vi "Create Palette File for VI Folder.vi"(5 "Include VIs in LLBs (T)":bool=TRUE, 6 "Filter Options":T1={"Exclude Dir Name pattern(s)"="^_", "Exclude LLB Name pattern(s)"="^_", "Exclude VI Name pattern(s)"="^_"}, 7 "Palette Icon":picture, 8 "error in":errorcluster, 9 "sub-palettes":path[](array[path]), 10 "Directory Path":path, 11 "Palette File in":path) -> (0 "error out":errorcluster, 2 "dup Directory Path":path, 3 "dup Palette File":path)   [LabVIEW 2014, in "VIHelpeksAPI.lvlib"]
doc: "::: VI Helpeks :::\nCopyright (c) 2000-2026 Konstantin Shifershteyn. All rights reserved."
uses:
  VIHelpeksAPI.lvlib
  <vilib>/Palette API/Palette Menu/Public Type Define/Palette Data.ctl
  <vilib>/Palette API/Palette Menu/Public Type Define/View Format.ctl
  <vilib>/Palette API/Palette Menu/Public Type Define/Items.ctl
  <vilib>/Palette API/Palette Menu/Public Type Define/Item.ctl
  <vilib>/Palette API/Palette Menu/Public Type Define/Help Info.ctl
  <vilib>/Palette API/Palette Menu/Public Type Define/Synchronize Info.ctl
  <vilib>/Palette API/Palette Menu/Public Type Define/Palette type.ctl
  <vilib>/Palette API/Palette Menu/Palette Menu.lvlib
panel:
  # "VI Helpeks\nCopyright (c) 2012-2026 Konstantin Shifershteyn"
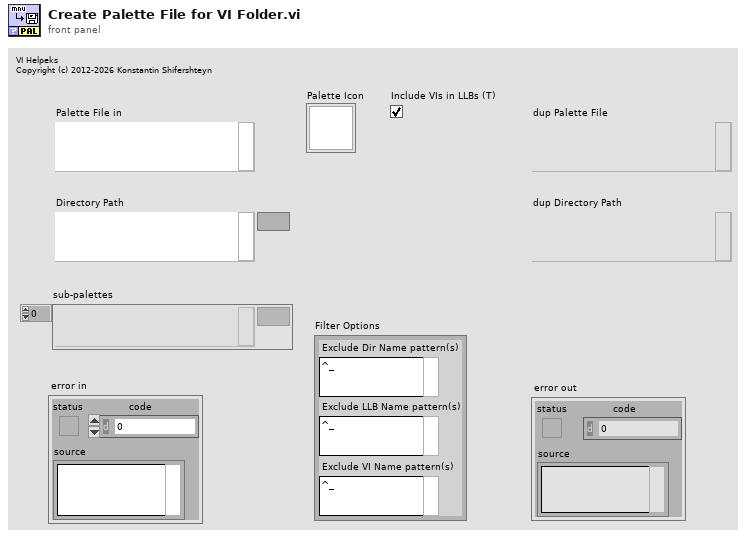
[diagram p1: front panel]
types:
  T1 = cluster{"Exclude Dir Name pattern(s)":string, "Exclude LLB Name pattern(s)":string, "Exclude VI Name pattern(s)":string}
  T2 = typedef "Palette Menu.lvlib/View Format.ctl" = u16
  T3 = typedef "Palette Menu.lvlib/Palette type.ctl" = i32
  T4 = typedef "Palette Menu.lvlib/Palette Data.ctl" = cluster{"display name":string, "view format":T2, "palette width":i16, "items":T5, "256 color icon":picture, "B&W color icon":picture, "help information":T7, "palette description":string, "synchronize information":T8}
  T5 = typedef "Palette Menu.lvlib/Items.ctl" = T6[]
  T6 = typedef "Palette Menu.lvlib/Item.ctl" = cluster{"item path":path, "library path (.lvlib)":path, "use default lvlib palette":bool, "short name":string, "place VI contents":bool, "hide synchronized item":bool, "reserve spot for synch item":bool, "configure when placing VI contents":bool}
  T7 = typedef "Palette Menu.lvlib/Help Info.ctl" = cluster{"help tag":string, "help file path ":path}
  T8 = typedef "Palette Menu.lvlib/Synchronize Info.ctl" = cluster{"synchronize with directory":bool, "synchronize directory path":path}
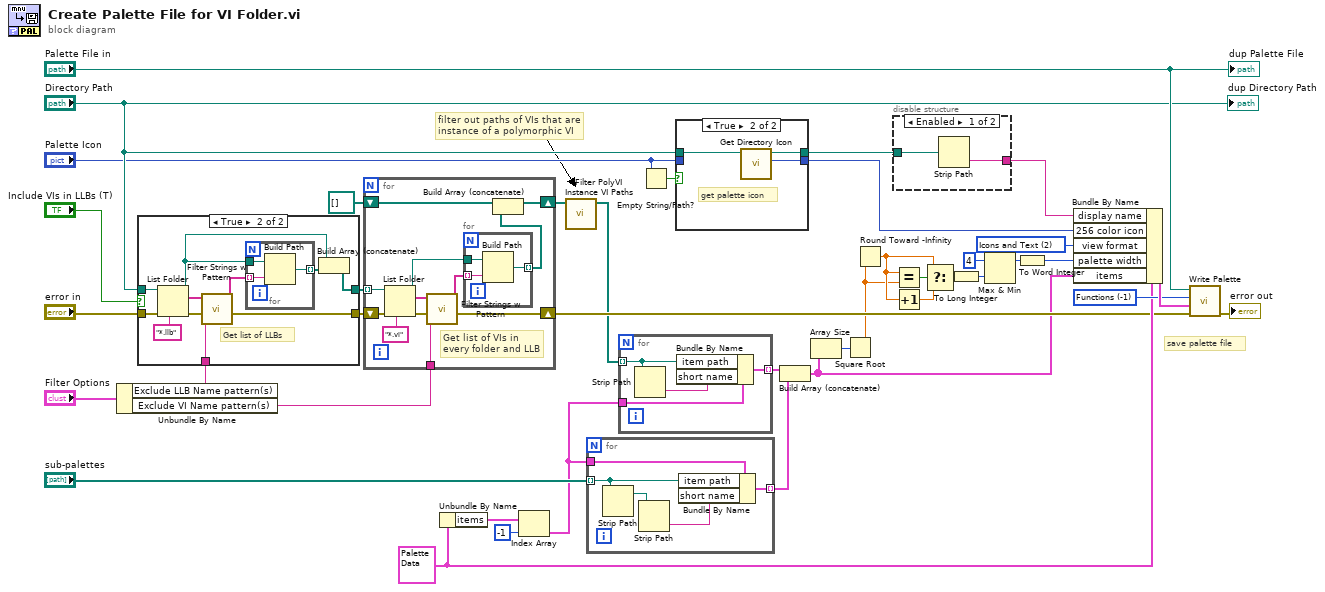
[diagram p0: block diagram]
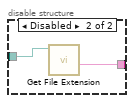
[diagram p3: hidden frame]
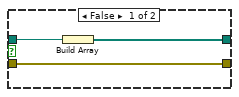
[diagram p4: hidden frame]
diagram:
  w38 = T2 2 items=["Icons", "Text", "Icons and Text"] ("view format")
  w39 = T3 -1 items=["Functions"=-1, "Controls"=-2] ("palette type")
  w37 = T4 {"display name"="", "view format"=2, "palette width"=4, "items"=[], "256 color icon"=bytes[0], "B&W color icon"=bytes[0], "help information"={"help tag"="", "help file path "=path ""}, "palette description"="", "synchronize information"={"synchronize with directory"=FALSE, "synchronize directory path"=path ""}} ("palette data")
  # "save palette file"
  # "filter out paths of VIs that are\ninstance of a polymorphic VI"
  n1 = Unbundle By Name("Filter Options") -> ("Exclude LLB Name pattern(s)"=w3:string, "Exclude VI Name pattern(s)"=w4:string)
  n2 = case shown="True" "Include VIs in LLBs (T)" {
    tunnel: "error in" -> [w43 w50]
    tunnel: [w43 w49] -> w22
    tunnel: "Directory Path" -> [w42 w47]
    tunnel: [w41 w46] -> w21
    tunnel: w3 -> [_ w44]
    frame False {
      n3 = Build Array(w42) -> (w41:path[])
    }
    frame True {
      # "Get list of LLBs"
      n4 = List Folder(path=w47, pattern="*.llb", error in=w50) -> (path out=w45:path, filenames=w52:string[], error out=w49:errorcluster)  [unwired: 1 in, 1 out]
      n5 = call "Filter Strings w Pattern.vi"("Exclude pattern(s) (^_)"=w44, "Array in"=w52) -> ("Array out"=w51:string[])  [unwired: 9 in]
      n6 = for {
        tunnel: w51 -> [w56] mode=indexing
        tunnel: w45 -> [w55]
        tunnel: [w54] -> w48 mode=indexing
        n7 = Build Path(base path=w55, name or relative path=w56) -> (appended path=w54:path)
      }
      n8 = Build Array (concatenate)(w45, w48) -> (w46:path[])
    }
  }
  n9 = for {
    shift-right: [w65] -> w30
    shift-left: w22 -> [w66]
    shift-right: [w62] -> w18
    shift-left: path[] [] -> [w63]
    tunnel: w21 -> [w61] mode=indexing
    tunnel: w4 -> [w57]
    # "Get list of VIs in\nevery folder and LLB"
    n10 = List Folder(path=w61, pattern="*.vi", error in=w66) -> (path out=w60:path, filenames=w64:string[], error out=w65:errorcluster)  [unwired: 1 in, 1 out]
    n11 = call "Filter Strings w Pattern.vi"("Exclude pattern(s) (^_)"=w57, "Array in"=w64) -> ("Array out"=w59:string[])  [unwired: 9 in]
    n12 = for {
      tunnel: w59 -> [w70] mode=indexing
      tunnel: w60 -> [w69]
      tunnel: [w68] -> w58 mode=indexing
      n13 = Build Path(base path=w69, name or relative path=w70) -> (appended path=w68:path)
    }
    n14 = Build Array (concatenate)(w63, w58) -> (w62:path[])
  }
  n15 = Unbundle By Name(w37) -> ("items"=w32:T5)
  n16 = Index Array(array=w32, index=-1) -> (element=w28:T6)
  n17 = call "Filter PolyVI Instance VI Paths.vi"("VI Paths"=w18) -> ("VI Paths out"=w17:path[])  [unwired: 10 in]
  n18 = for {
    tunnel: w28 -> [w75]
    tunnel: [w74] -> w26 mode=indexing
    tunnel: "sub-palettes" -> [w73] mode=indexing
    n19 = Strip Path(path=w73) -> (stripped path=w72:path)  [unwired: 1 out]
    n20 = Strip Path(path=w72) -> (name=w71:string)  [unwired: 1 out]
    n21 = Bundle By Name(cluster=w75, "item path"=w73, "short name"=w71) -> (w74:T6)
  }
  n22 = for {
    tunnel: w28 -> [w79]
    tunnel: w17 -> [w77] mode=indexing
    tunnel: [w78] -> w36 mode=indexing
    n23 = Strip Path(path=w77) -> (name=w76:string)  [unwired: 1 out]
    n24 = Bundle By Name(cluster=w79, "item path"=w77, "short name"=w76) -> (w78:T6)
  }
  n25 = Empty String/Path?(string/path="Palette Icon") -> (empty?=w2:bool)
  n26 = case shown="True" w2 {
    tunnel: "Directory Path" -> [w81 w84]
    tunnel: [w80 w83] -> w8
    tunnel: [w81 w82] -> w6
    tunnel: "Palette Icon" -> [w80 _]
    frame False {
    }
    frame True {
      # "get palette icon"
      n27 = call "Get Directory Icon.vi"("Directory Path"=w84) -> ("Icon"=w83:picture, "dup Directory Path"=w82:path)  [unwired: 8 in, 1 out]
    }
  }
  n28 = Build Array (concatenate)(w36, w26) -> (w27:T6[])
  n29 = Array Size(array=w27) -> (size(s)=w10:i32)
  n30 = Square Root(x=w10) -> (sqrt(x)=w12:dbl)
  n31 = Round Toward -Infinity(1:w12) -> (0:w14:dbl)
  n32 = disable-structure shown="Enabled" {
    disable-tunnel: w6 -> [w86 w88]
    disable-tunnel: [w85 w87] -> w7
    frame Enabled {
      n33 = Strip Path(path=w86) -> (name=w85:string)  [unwired: 1 out]
    }
    frame Disabled {
      n34 = call <vilib>:"Get File Extension.vi"("file"=w88) -> ("filename without extension"=w87:string)  [unwired: 7 in, 3 out]
    }
  }
  n35 = Equal?(x=w14, y=w12) -> (x = y?=w13:bool)
  n36 = Increment(x=w14) -> (x+1=w15:dbl)
  n37 = Select(t=w14, s=w13, f=w15) -> (s? t:f=w16:dbl)
  n38 = To Long Integer(number=w16) -> (32bit integer=w11:i32)
  n39 = Max & Min(x=4, y=w11) -> (max(x,y)=w34:i32)  [unwired: 1 out]
  n40 = To Word Integer(number=w34) -> (16bit integer=w25:i16)
  n41 = Bundle By Name(cluster=w37, "display name"=w7, "256 color icon"=w8, "view format"=w38, "palette width"=w25, "items"=w27) -> (w40:T4)
  n42 = call <vilib>:"Write Palette.vi"("error in (no error)"=w30, "palette data"=w40, "palette type"=w39, "palette path"="Palette File in") -> ("error out"=→"error out":errorcluster)  [unwired: 7 in]
  "dup Palette File" <- "Palette File in"
  "dup Directory Path" <- "Directory Path"
